vi "U8 Array to CAN Display.vi"(8 "error in (no error)":errorcluster, 11 "U8 Array":T1 {"u8_array"."u8_array" format="%.0x"}) -> (0 "error out":errorcluster, 3 "CAN Data for Mutli Listbox":string[][](array[string]))   [LabVIEW 2021, in "CIF CAN_Reader_CANsub UI.lvlib"]
uses:
  CIF CAN_Reader_CANsub UI.lvlib
  <vilib>/CIF Foundation/CIF U8 Array Monitor gRPC/U8_Array_Monitor_gRPC/CIFU8ArrayMonitor_client/RPC Messages/cif_u8arraymonitor_U8Arrays.ctl
  <vilib>/CIF Foundation/CIF U8 Array Monitor gRPC/U8_Array_Monitor_gRPC/CIFU8ArrayMonitor_client/RPC Messages/cif_u8arraymonitor_U8Array.ctl
  <vilib>/CIF Foundation/CIF XNET CAN RW/typedef/CAN Return Map.ctl
  <vilib>/xnet/xnet.llb/XNET Frame CAN.ctl
  <vilib>/xnet/xnet.llb/XNET Frame Type CAN.ctl
  <vilib>/CIF Foundation/CIF XNET CAN RW/Utilities/Unflatten pcap CAN to XNET CAN.vi
  <vilib>/CIF Foundation/CIF XNET CAN RW/XNET CAN RW.lvclass
  <vilib>/CIF Foundation/CIF U8 Array Monitor gRPC/U8_Array_Monitor_gRPC/CIFU8ArrayMonitor_client/CIFU8ArrayMonitor_client.lvlib
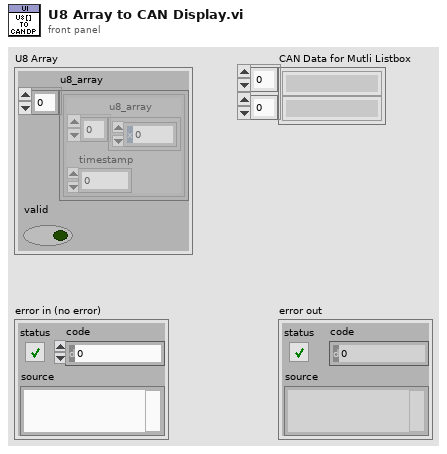
[diagram p1: front panel]
types:
  T1 = typedef "CIFU8ArrayMonitor_client.lvlib/cif_u8arraymonitor_U8Arrays.ctl" = cluster{"u8_array":T2[], "valid":bool}
  T2 = typedef "CIFU8ArrayMonitor_client.lvlib/cif_u8arraymonitor_U8Array.ctl" = cluster{"u8_array":u8[], "timestamp":i64}
  T3 = typedef "XNET CAN RW.lvclass/CAN Return Map.ctl" = map{u32, T4}
  T4 = typedef "XNET Frame CAN.ctl" = cluster{"timestamp":timestamp, "payload":u8[], "identifier":u32, "type":T5, "extended?":bool, "echo?":bool}
  T5 = typedef "XNET Frame Type CAN.ctl" = u8
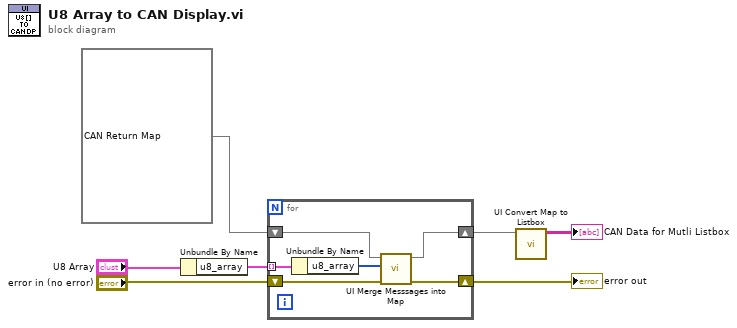
[diagram p0: block diagram]
diagram:
  n1 = Unbundle By Name("U8 Array") -> ("u8_array"=w5:T2[])
  n2 = for {
    tunnel: w5 -> [w13] mode=indexing
    shift-right: [w11] -> w7
    shift-left: "error in (no error)" -> [w12]
    shift-right: [w8] -> w2
    shift-left: T3 {} ("CAN Return MAP in") -> [w9]
    n3 = Unbundle By Name(w13) -> ("u8_array"=w10:u8[])
    n4 = call <vilib>:"UI Merge Messsages into Map.vi"("error in (no error)"=w12, "pcap CAN DATA in"=w10, "CAN Return MAP in"=w9) -> ("error out"=w11:errorcluster, "CAN Return MAP out"=w8:T3)  [unwired: 7 in]
  }
  "error out" <- w7
  n5 = call <vilib>:"UI Convert Map to Listbox.vi"("CAN Return MAP in"=w2) -> ("CAN Data for Mutli Listbox"=→"CAN Data for Mutli Listbox":string[][])  [unwired: 10 in]
